vi "Config.vi"(8 "error in (no error)":errorcluster, 10 "Setting":variant, 11 "Tektronix Scope in":refnum<class "Tektronix MSO5.lvclass">) -> (0 "error out":errorcluster, 3 "Tektronix Scope out":refnum<class "Tektronix MSO5.lvclass">)   [LabVIEW 2025, in "Scope.lvlib" / "Tektronix MSO5.lvclass"]
uses:
  Tektronix MSO5.lvclass
  C:/Working copy/TS Manager/Plugin/Engines/Scope/Scope Instrument/Scope Instrument.lvclass
  C:/Users/Public/Documents/Sandia National Labs/TSS Plugin/CEF.lvlibp/Node/CEF_Node.lvclass
  C:/Users/Public/Documents/Sandia National Labs/TSS Plugin/Abstract Engine.lvlibp/Abstract Instrument/Abstract Instrument.lvclass
  Scope Channel/Scope Channel.lvclass
  Scope configuration/Scope configuration.lvclass
  Tektronix MSO5.lvclass/Tektronix MSO5.ctl
  Scope configuration/Scope configuration.lvclass/Scope configuration.ctl
  <instrlib>/niScope/Controls/niScope trigger coupling.ctl
  Users/Public/Documents/Sandia National Labs/TSS Plugin/Abstract Engine.lvlibp/Abstract Instrument/Channel.ctl
  Users/Public/Documents/Sandia National Labs/TSS Plugin/Abstract Engine.lvlibp/Abstract Instrument/Data Type.ctl
  Scope Channel configuration/Scope Channel configuration.lvclass
  C:/Users/Public/Documents/Sandia National Labs/TSS Plugin/Abstract Engine.lvlibp/Channel configuration/Channel configuration.lvclass
  Scope Channel configuration/Scope Channel configuration.lvclass/Scope Channel configuration.ctl
  <instrlib>/niScope/Controls/niScope vertical coupling.ctl
  Scope Channel configuration/Read Scope Channel.vi
  Scope configuration/Read Scope Setting.vi
  Users/Public/Documents/Sandia National Labs/TSS Plugin/CEF.lvlibp/Node/ReadChildren.vi
  Users/Public/Documents/Sandia National Labs/TSS Plugin/Abstract Engine.lvlibp/Channel configuration/Read Channel Setting.vi
  <instrlib>/Tektronix MSO5X Series/Public/Configure/Configure Trigger (A Mode).vi
  Users/Public/Documents/Sandia National Labs/TSS Plugin/CEF.lvlibp/serializable configuration/CEF_serializable configuration.lvclass
  Users/Public/Documents/Sandia National Labs/TSS Plugin/CEF.lvlibp/Node/CEF_Node.lvclass
  Users/Public/Documents/Sandia National Labs/TSS Plugin/Abstract Engine.lvlibp/Abstract Instrument/Abstract Instrument.lvclass
  <instrlib>/Tektronix MSO5X Series/Tektronix MSO5X Series.lvlib
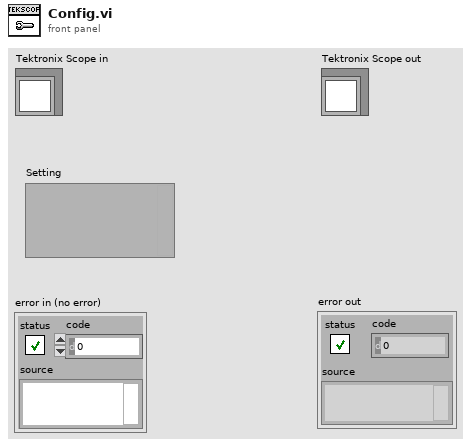
[diagram p1: front panel]
types:
  T1 = typedef "Abstract Engine.lvlibp/Abstract Instrument.lvclass/Channel.ctl" = cluster{"Alias":string, "DataType":T2, "Unit":enum16{"---", "V", "A", "Ohm", "Hz", "uF", "degC", "deg"}, "Upper limit":dbl, "Lower limit":dbl, "Measurement":variant}
  T2 = typedef "Abstract Engine.lvlibp/Abstract Instrument.lvclass/Data Type.ctl" = string
  T3 = typedef "Abstract Engine.lvlibp/Channel configuration.lvclass/Default Channel.ctl" = cluster{"Address":string, "SW Alias":string, "Enabled":bool, "Type":string, "Description":string}
  T4 = typedef "Scope.lvlib/Scope Channel configuration.lvclass/Scope Channel Setting.ctl" = cluster{"Gain":u32, "Offset":u32, "Vertical Range":dbl, "Vertical Offset":dbl, "Unit":string, "Attenuation":dbl, "Vertical Coupling":string, "Impedance":string, "Auto Setup":bool}
  T5 = typedef "niScope vertical coupling.ctl" = i32
  T6 = typedef "Scope.lvlib/Scope configuration.lvclass/Scope Instrument Setting.ctl" = cluster{"Sampling Rate":dbl, "Number of Samples":u32, "Type":string, "Source":string, "Trigger Coupling":string, "TrigDest":string, "Group":string, "Pretrigger":dbl, "Level 1":dbl, "Level 2":dbl}
  T7 = typedef "niScope trigger coupling.ctl" = u16
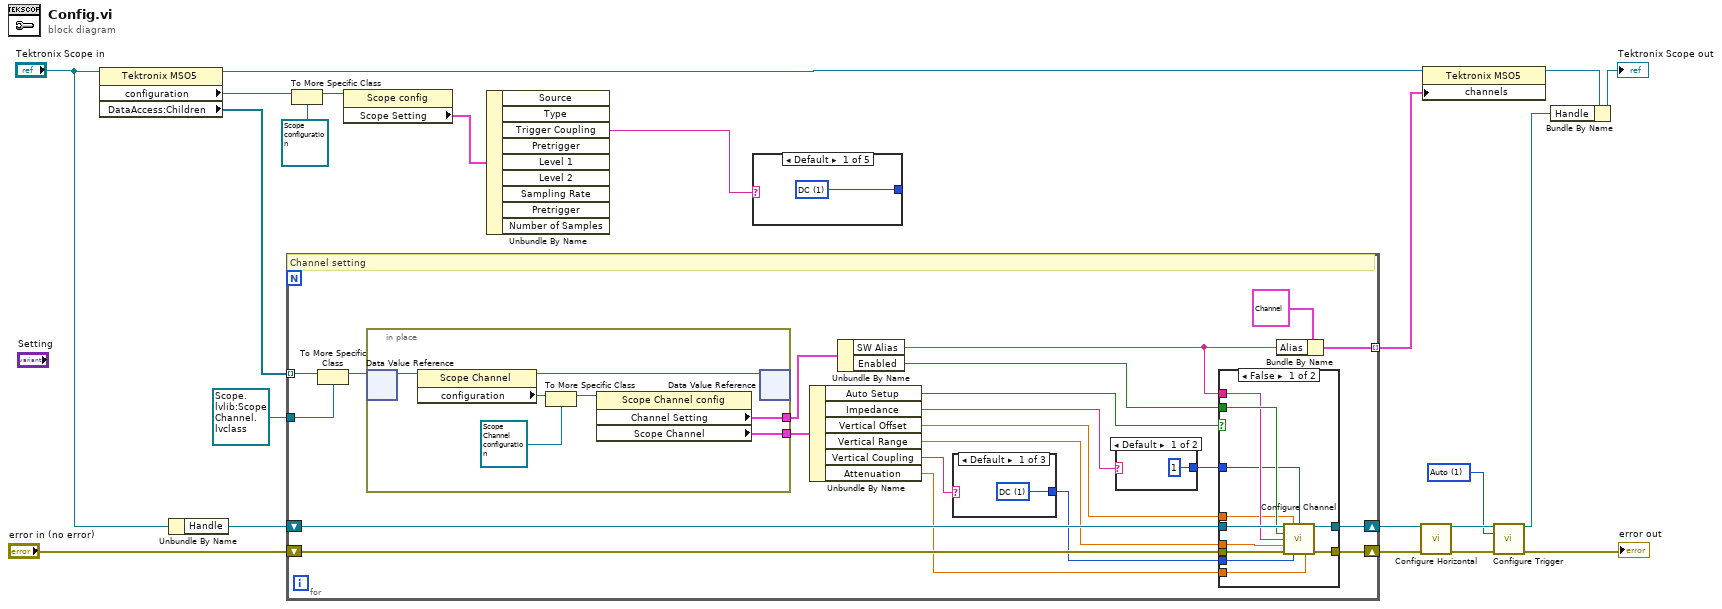
[diagram p0: block diagram]
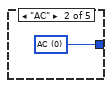
[diagram p2: hidden frame]
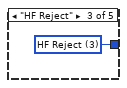
[diagram p3: hidden frame]
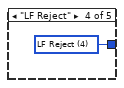
[diagram p4: hidden frame]
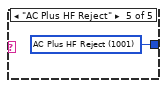
[diagram p5: hidden frame]
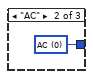
[diagram p6: hidden frame]
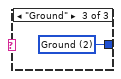
[diagram p7: hidden frame]
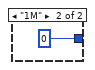
[diagram p8: hidden frame]
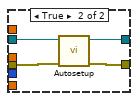
[diagram p9: hidden frame]
diagram:
  w1 = u16 1 items=["Normal", "Auto"] ("Trigger Mode (1:Auto)")
  n1 = property class="Tektronix MSO5"(reference="Tektronix Scope in") -> (reference out=w19:refnum<class "Tektronix MSO5.lvclass">, "configuration"=w16:refnum<class "CEF_serializable configuration.lvclass">, "DataAccess:Children"=w14:refnum<data-value>[])  [unwired: 1 in, 1 out]
  n2 = Unbundle By Name("Tektronix Scope in") -> ("Handle"=w17:refnum<visa-resource-name>)
  n3 = for {
    tunnel: [w29] -> w8 mode=indexing
    shift-right: [w36] -> w5
    shift-left: "error in (no error)" -> [w38]
    shift-right: [w37] -> w4
    shift-left: w17 -> [w39]
    tunnel: w14 -> [w42] mode=indexing
    tunnel: refnum<data-value> refnum ("data value reference") -> [w40]
    # "Channel setting"
    n4 = To More Specific Class(target class=w40, reference=w42) -> (specific class reference=w41:refnum<data-value>)  [unwired: 1 in, 1 out]
    n5 = in-place {
      in-place-border: [w44] -> w35
      in-place-border: [w43] -> w33
      # "Initialize the front panel controls when loaded"
      n6 = in-place-dvr #1(w41) -> (w49:refnum<class "Scope Channel.lvclass">)  [unwired: 1 out]
      n7 = property class="Scope Channel"(reference=w49) -> (reference out=w48:refnum<class "Scope Channel.lvclass">, "configuration"=w47:refnum<class "CEF_serializable configuration.lvclass">)  [unwired: 1 in, 1 out]
      n8 = To More Specific Class(target class=refnum<class "Scope Channel configuration.lvclass"> refnum ("Scope.lvlib:Scope Channel configuration.lvclass"), reference=w47) -> (specific class reference=w46:refnum<class "Scope Channel configuration.lvclass">)  [unwired: 1 in, 1 out]
      n9 = property class="Scope Channel config"(reference=w46) -> ("Channel Setting"=w44:T3, "Scope Channel"=w43:T4)  [unwired: 1 in, 2 out]
      n10 = in-place-dvr #1(w48) -> ()  [unwired: 2 out]
    }
    n11 = Unbundle By Name(w33) -> ("Auto Setup"=w32:bool, "Impedance"=w22:string, "Vertical Offset"=w25:dbl, "Vertical Range"=w26:dbl, "Vertical Coupling"=w31:string, "Attenuation"=w23:dbl)
    n12 = Unbundle By Name(w35) -> ("SW Alias"=w30:string, "Enabled"=w34:bool)
    n13 = case shown="Default" w31 {
      tunnel: [w50 w51 w52] -> w27
      frame Default {
        w50 = T5 1 items=["AC", "DC", "Ground"] ("Coupling")
      }
      frame "AC" {
        w51 = T5 0 items=["AC", "DC", "Ground"] ("Coupling")
      }
      frame "Ground" {
        w52 = T5 2 items=["AC", "DC", "Ground"] ("Coupling")
      }
    }
    n14 = case shown="Default" w22 {
      tunnel: [u32 1 ("Impedance") u32 0 ("Impedance")] -> w24
      frame Default {
      }
      frame "1M" {
      }
    }
    n15 = case shown="False" w32 {
      tunnel: w39 -> [w65 w69]
      tunnel: [w64 w68] -> w37
      tunnel: w38 -> [w62 w67]
      tunnel: [w63 w66] -> w36
      tunnel: w30 -> [w60 _]
      tunnel: w34 -> [w61 _]
      tunnel: w23 -> [w59 _]
      tunnel: w27 -> [w58 _]
      tunnel: w26 -> [w57 _]
      tunnel: w25 -> [w56 _]
      tunnel: w24 -> [w55 _]
      frame False {
        n16 = call <instrlib>:"Configure Channel.vi"("VISA resource name"=w65, "Vertical Offset (0.0 V)"=w56, "Input Impedance (0: 1M ohm)"=w55, "Enable Channel (T: Enable)"=w61, "Channel (CH1)"=w60, "Vertical Range (10.0 V)"=w57, "error in (no error)"=w62, "Vertical Coupling (1: DC)"=w58, "Net Attenuation (1.0)"=w59) -> ("VISA resource name out"=w64:refnum<visa-resource-name>, "error out"=w63:errorcluster)  [unwired: 5 in]
      }
      frame True {
        n17 = call <instrlib>:"Autosetup.vi"("error in (no error)"=w67, "VISA resource name"=w69) -> ("error out"=w66:errorcluster, "VISA resource name out"=w68:refnum<visa-resource-name>)  [unwired: 8 in]
      }
    }
    n18 = Bundle By Name(cluster=T1 {"Alias"="ch0", "DataType"="Analog Input", "Unit"=enum."V", "Upper limit"=10.0, "Lower limit"=-10.0, "Measurement"=variant} ("Channel"), "Alias"=w30) -> (w29:T1)
  }
  n19 = To More Specific Class(target class=refnum<class "Scope configuration.lvclass"> refnum ("Scope.lvlib:Scope configuration.lvclass"), reference=w16) -> (specific class reference=w15:refnum<class "Scope configuration.lvclass">)  [unwired: 1 in, 1 out]
  n20 = property class="Scope config"(reference=w15) -> ("Scope Setting"=w10:T6)  [unwired: 1 in, 2 out]
  n21 = Unbundle By Name(w10) -> ("Trigger Coupling"=w11:string)  [unwired: 8 out]
  n22 = case shown="Default" w11 {
    tunnel: [w70 w71 w72 w73 w74] -> _
    frame Default {
      w70 = T7 1 items=["AC"=0, "DC"=1, "HF Reject"=3, "LF Reject"=4, "AC Plus HF Reject"=1001] ("Trigger Coupling")
    }
    frame "AC" {
      w71 = T7 0 items=["AC"=0, "DC"=1, "HF Reject"=3, "LF Reject"=4, "AC Plus HF Reject"=1001] ("Trigger Coupling")
    }
    frame "HF Reject" {
      w72 = T7 3 items=["AC"=0, "DC"=1, "HF Reject"=3, "LF Reject"=4, "AC Plus HF Reject"=1001] ("Trigger Coupling")
    }
    frame "LF Reject" {
      w73 = T7 4 items=["AC"=0, "DC"=1, "HF Reject"=3, "LF Reject"=4, "AC Plus HF Reject"=1001] ("Trigger Coupling")
    }
    frame "AC Plus HF Reject" {
      w74 = T7 1001 items=["AC"=0, "DC"=1, "HF Reject"=3, "LF Reject"=4, "AC Plus HF Reject"=1001] ("Trigger Coupling")
    }
  }
  n23 = call <instrlib>:"Configure Horizontal.vi"("VISA resource name"=w4, "error in (no error)"=w5) -> ("VISA resource name out"=w7:refnum<visa-resource-name>, "error out"=w6:errorcluster)  [unwired: 12 in]
  n24 = property class="Tektronix MSO5"(reference=w19, "channels"=w8) -> (reference out=w9:refnum<class "Tektronix MSO5.lvclass">)  [unwired: 1 in, 1 out]
  n25 = call-poly <instrlib>:"Configure Trigger.vi"("VISA resource name"=w7, "Trigger Mode (1:Auto)"=w1, "error in (no error)"=w6) -> ("VISA resource name out"=w2:refnum<visa-resource-name>, "error out"=→"error out":errorcluster)  [unwired: 11 in]
  n26 = Bundle By Name(cluster=w9, "Handle"=w2) -> (→"Tektronix Scope out":refnum<class "Tektronix MSO5.lvclass">)
